vi "TurnTable Loop.vi"(8 "error in (no error)":errorcluster caption="에러 입력(에러 없음)", 10 "Sad Queue":refnum<queue>, 11 "Instrument Manager 입력":refnum<class "Instrument Manager.lvclass">) -> (0 "error out":errorcluster caption="에러 출력", 3 "Instrument Manager 출력":refnum<class "Instrument Manager.lvclass">)   [LabVIEW 2023, in "Instrument Manager.lvclass"]
uses:
  Instrument Manager.lvclass
  Instrument Manager.lvclass/Instrument Manager.ctl
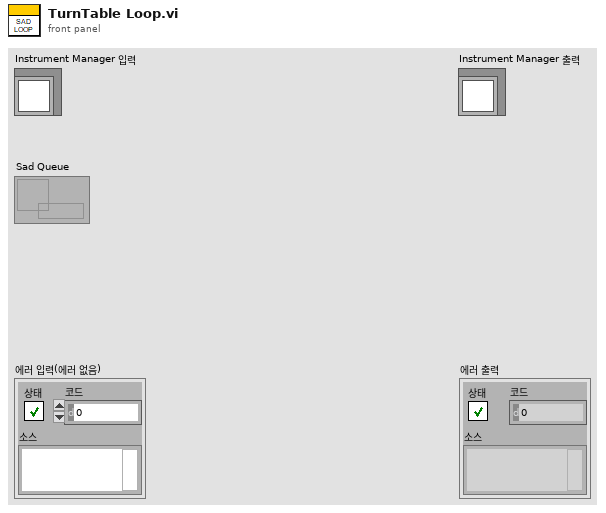
[diagram p1: front panel]
types:
  T1 = cluster{"Turn Table Info":cluster{"Target Angle":dbl, "Turn Table Speed":i32, "Fetch Interval":i32}, "Instrument Manager 입력":refnum<class "Instrument Manager.lvclass">}
  T2 = cluster{"Target Angle":dbl, "Turn Table Speed":i32, "Fetch Interval":i32}
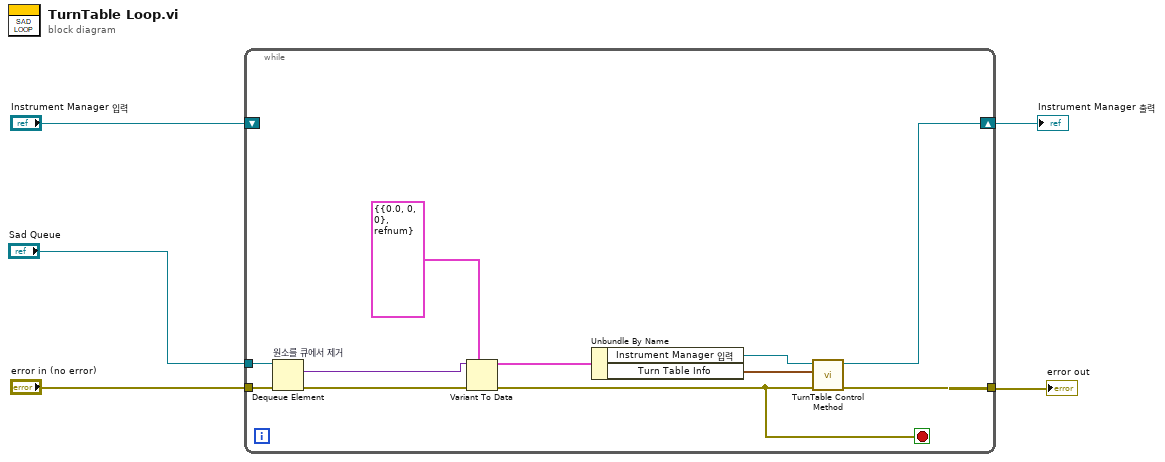
[diagram p0: block diagram]
diagram:
  n1 = while {
    shift-right: [w14] -> w2
    shift-left: "Instrument Manager 입력" -> [_]
    tunnel: "Sad Queue" -> [w11]
    tunnel: "error in (no error)" -> [w16]
    tunnel: [w15] -> w3
    stop <- w6 stop-if-true
    n2 = Dequeue Element "원소를 큐에서 제거"(queue=w11, error in (no error)=w16) -> (element=w9:variant, error out=w10:errorcluster)  [unwired: 1 in, 2 out]
    n3 = Variant To Data(error in=w10, type=T1 {"Turn Table Info"={"Target Angle"=0.0, "Turn Table Speed"=0, "Fetch Interval"=0}, "Instrument Manager 입력"=refnum} ("원소"), Variant=w9) -> (data=w7:T1, error out=w6:errorcluster)
    n4 = Unbundle By Name(w7) -> ("Instrument Manager 입력"=w13:refnum<class "Instrument Manager.lvclass">, "Turn Table Info"=w12:T2)
    n5 = call "TurnTable Control Method.vi"("error in (no error)"=w6, "Turn Table Info"=w12, "Instrument Manager 입력"=w13) -> ("error out"=w15:errorcluster, "Instrument Manager 출력"=w14:refnum<class "Instrument Manager.lvclass">)  [unwired: 7 in]
  }
  "error out" <- w3
  "Instrument Manager 출력" <- w2
